vi "Data-DCSL__RecursionCtl.vi"(8 "TEMP DONT LINE":cluster{"LabelPath":string, "Ref":refnum<vi>}[](array[cluster]), 11 "Controls[] input":cluster{"LabelPath":string, "Ref":refnum<vi>}[](array[cluster])) -> (3 "Controls[] output":cluster{"LabelPath":string, "Ref":refnum<vi>}[](array[cluster]))   [LabVIEW 2017]
doc: "<B>#yyll</B>\nGetAllRefsByRecursion"
panel:
  # "递归了\nRadio Buttons（感觉没必要）\nCluster\nTab Control\n\n没递归\n数组"
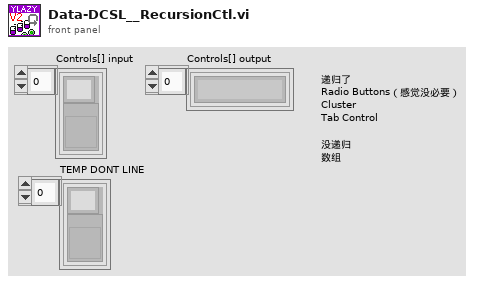
[diagram p1: front panel]
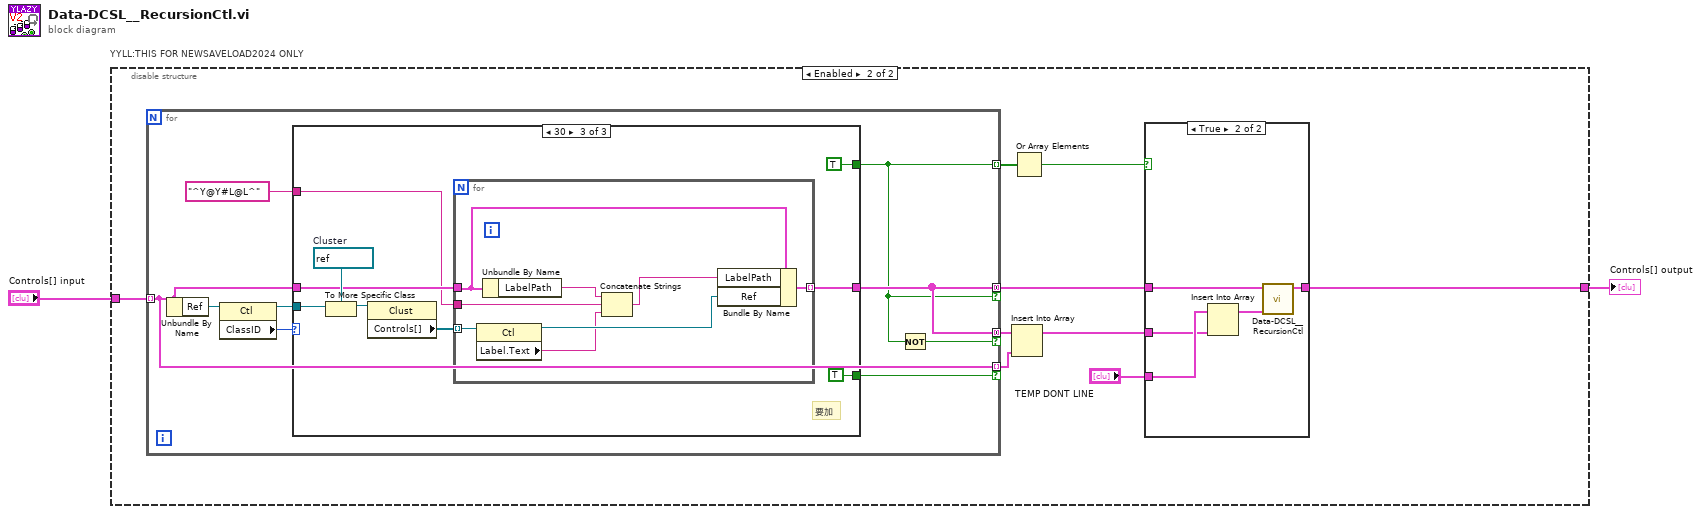
[diagram p0: block diagram]
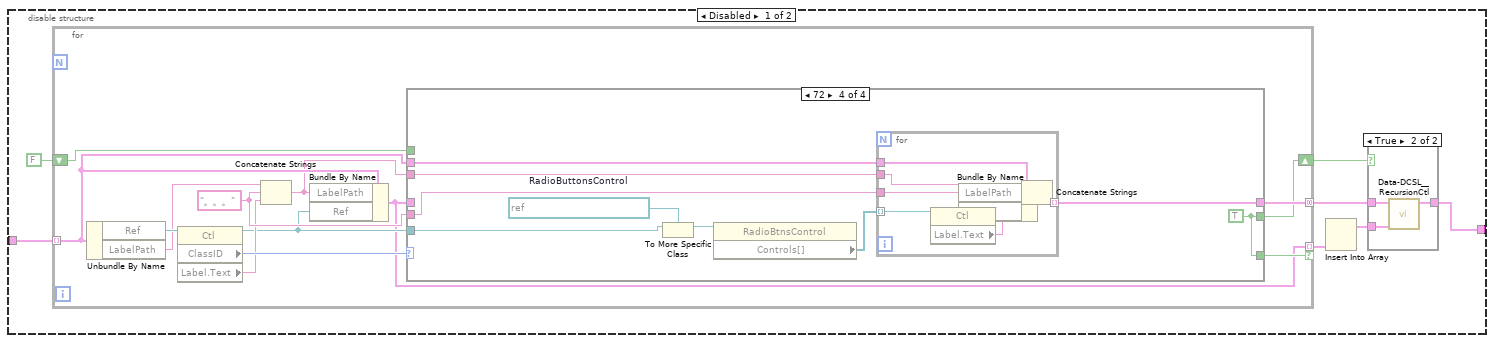
[diagram p2: hidden frame]
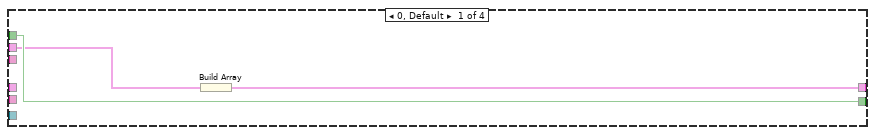
[diagram p3: hidden frame]
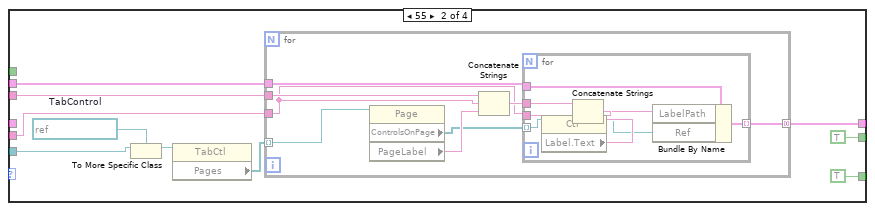
[diagram p4: hidden frame]
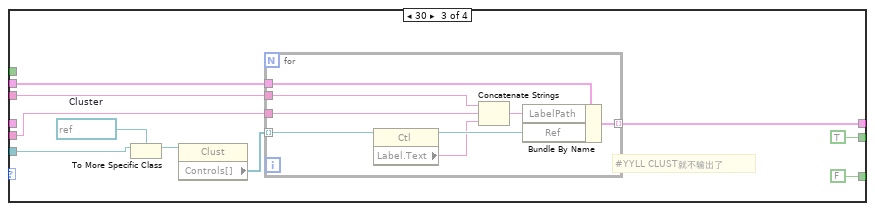
[diagram p5: hidden frame]
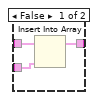
[diagram p6: hidden frame]
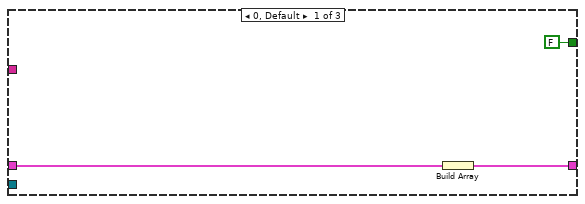
[diagram p7: hidden frame]
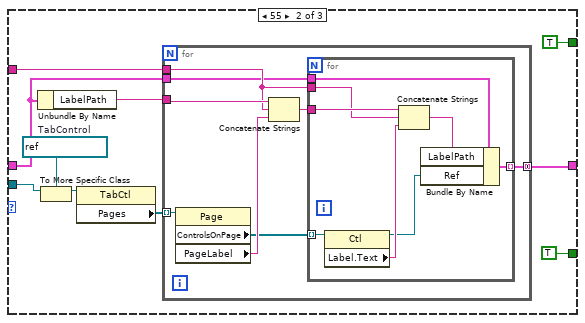
[diagram p8: hidden frame]
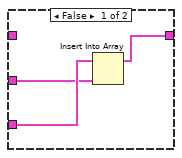
[diagram p9: hidden frame]
diagram:
  n1 = disable-structure "YYLL:THIS FOR NEWSAVELOAD2024 ONLY" shown="Enabled" {
    disable-tunnel: [w9 w97] -> w2
    disable-tunnel: "Controls[] input" -> [w8 w101]
    frame Disabled {
      n2 = for {
        tunnel: [w22] -> w7 mode=concatenating
        tunnel: w8 -> [w13] mode=indexing
        tunnel: [w11] -> w3 mode=indexing if=w18
        shift-right: [w21] -> w4
        shift-left: FALSE -> [w20]
        w15 = "。。。" ("string")
        n3 = Unbundle By Name(w13) -> ("Ref"=w17:refnum<vi>, "LabelPath"=w16:string)
        n4 = property class="Ctl"(reference=w17) -> (reference out=w12:refnum<vi>, "ClassID"=w19:u32, "Label.Text"=w14:string)  [unwired: 1 in, 1 out]
        n5 = Concatenate Strings(w16, w15, w14) -> (w10:string)
        n6 = Bundle By Name(cluster=w13, "LabelPath"=w10, "Ref"=w12) -> (w11:cluster{"LabelPath":string, "Ref":refnum<vi>})
        n7 = case shown="72" w19 {
          tunnel: w12 -> [_ w32 w60 w76]
          tunnel: [w25 w31 w54 w71] -> w22
          tunnel: [w24 TRUE TRUE w78] -> w21
          tunnel: w20 -> [w24 _ _ _]
          tunnel: [_ TRUE FALSE w78] -> w18
          tunnel: w13 -> [w23 w28 w56 w73]
          tunnel: w15 -> [_ w29 w55 w72]
          tunnel: w11 -> [_ _ _ _]
          tunnel: w10 -> [_ w26 w52 w70]
          frame 0, Default {
            n8 = Build Array(w23) -> (w25:cluster{"LabelPath":string, "Ref":refnum<vi>}[])
          }
          frame 55 {
            w35 = refnum<vi> refnum  # TabControl
            n9 = To More Specific Class(target class=w35, reference=w32) -> (specific class reference=w34:refnum<vi>)  [unwired: 1 in, 1 out]
            n10 = property class="TabCtl"(reference=w34) -> ("Pages"=w33:refnum<vi>[])  [unwired: 1 in, 2 out]
            n11 = for {
              tunnel: w33 -> [w43] mode=indexing
              tunnel: [w36] -> w31 mode=concatenating
              tunnel: w26 -> [w42]
              tunnel: w29 -> [w38]
              tunnel: w28 -> [w37]
              n12 = property class="Page"(reference=w43) -> ("ControlsOnPage"=w40:refnum<vi>[], "PageLabel"=w41:string)  [unwired: 1 in, 2 out]
              n13 = Concatenate Strings(w42, w38, w41) -> (w39:string)
              n14 = for {
                tunnel: w40 -> [w51] mode=indexing
                tunnel: w39 -> [w49]
                tunnel: w38 -> [w48]
                tunnel: w37 -> [w47]
                tunnel: [w44] -> w36 mode=indexing
                n15 = property class="Ctl"(reference=w51) -> (reference out=w45:refnum<vi>, "Label.Text"=w50:string)  [unwired: 1 in, 1 out]
                n16 = Concatenate Strings(w49, w48, w50) -> (w46:string)
                n17 = Bundle By Name(cluster=w47, "LabelPath"=w46, "Ref"=w45) -> (w44:cluster{"LabelPath":string, "Ref":refnum<vi>})
              }
            }
          }
          frame 30 {
            w61 = refnum<vi> refnum  # Cluster
            # "#YYLL CLUST就不输出了"
            n18 = To More Specific Class(target class=w61, reference=w60) -> (specific class reference=w59:refnum<vi>)  [unwired: 1 in, 1 out]
            n19 = property class="Clust"(reference=w59) -> ("Controls[]"=w57:refnum<vi>[])  [unwired: 1 in, 2 out]
            n20 = for {
              tunnel: w57 -> [w68] mode=indexing
              tunnel: w56 -> [w69]
              tunnel: w52 -> [w66]
              tunnel: w55 -> [w65]
              tunnel: [w62] -> w54 mode=indexing
              n21 = property class="Ctl"(reference=w68) -> (reference out=w64:refnum<vi>, "Label.Text"=w63:string)  [unwired: 1 in, 1 out]
              n22 = Concatenate Strings(w66, w65, w63) -> (w67:string)
              n23 = Bundle By Name(cluster=w69, "LabelPath"=w67, "Ref"=w64) -> (w62:cluster{"LabelPath":string, "Ref":refnum<vi>})
            }
          }
          frame 72 {
            w77 = refnum<vi> refnum  # RadioButtonsControl
            w78 = TRUE
            n24 = To More Specific Class(target class=w77, reference=w76) -> (specific class reference=w75:refnum<vi>)  [unwired: 1 in, 1 out]
            n25 = property class="RadioBtnsControl"(reference=w75) -> ("Controls[]"=w74:refnum<vi>[])  [unwired: 1 in, 2 out]
            n26 = for {
              tunnel: w74 -> [w85] mode=indexing
              tunnel: w73 -> [w86]
              tunnel: w70 -> [w83]
              tunnel: w72 -> [w82]
              tunnel: [w79] -> w71 mode=indexing
              n27 = property class="Ctl"(reference=w85) -> (reference out=w81:refnum<vi>, "Label.Text"=w80:string)  [unwired: 1 in, 1 out]
              n28 = Concatenate Strings(w83, w82, w80) -> (w84:string)
              n29 = Bundle By Name(cluster=w86, "LabelPath"=w84, "Ref"=w81) -> (w79:cluster{"LabelPath":string, "Ref":refnum<vi>})
            }
          }
        }
      }
      n30 = Insert Into Array(new element=w3) -> (w6:cluster{"LabelPath":string, "Ref":refnum<vi>}[])  [unwired: 2 in]
      n31 = case shown="True" w4 {
        tunnel: w7 -> [w89 w92]
        tunnel: [w88 w91] -> w9
        tunnel: w6 -> [w87 w90]
        frame False {
          n32 = Insert Into Array(array=w89, new element=w87) -> (w88:cluster{"LabelPath":string, "Ref":refnum<vi>}[])  [unwired: 1 in]
        }
        frame True {
          n33 = call "Data-DCSL__RecursionCtl.vi"("TEMP DONT LINE"=w90, "Controls[] input"=w92) -> ("Controls[] output"=w91:cluster{"LabelPath":string, "Ref":refnum<vi>}[])  [unwired: 9 in]
        }
      }
    }
    frame Enabled {
      n34 = for {
        tunnel: w101 -> [w103] mode=indexing
        tunnel: [w106] -> w100 mode=indexing
        tunnel: [w107] -> w98 mode=concatenating if=w106
        tunnel: [w107] -> w95 mode=concatenating if=w105
        tunnel: [w103] -> w93 mode=indexing if=w102
        n35 = Unbundle By Name(w103) -> ("Ref"=w110:refnum<vi>)
        n36 = property class="Ctl"(reference=w110) -> (reference out=w108:refnum<vi>, "ClassID"=w109:u32)  [unwired: 1 in, 1 out]
        n37 = case shown="30" w109 {
          tunnel: w108 -> [_ w120 w145]
          tunnel: [FALSE TRUE TRUE] -> w106
          tunnel: w103 -> [w112 w116 w143]
          tunnel: [w111 w115 w141] -> w107
          tunnel: "^Y@Y#L@L^" ("string") -> [_ w117 w142]
          tunnel: [_ TRUE TRUE] -> w102
          frame 0, Default {
            n38 = Build Array(w112) -> (w111:cluster{"LabelPath":string, "Ref":refnum<vi>}[])
          }
          frame 55 {
            w121 = refnum<vi> refnum  # TabControl
            n39 = Unbundle By Name(w116) -> ("LabelPath"=w118:string)
            n40 = To More Specific Class(target class=w121, reference=w120) -> (specific class reference=w122:refnum<vi>)  [unwired: 1 in, 1 out]
            n41 = property class="TabCtl"(reference=w122) -> ("Pages"=w119:refnum<vi>[])  [unwired: 1 in, 2 out]
            n42 = for {
              tunnel: w119 -> [w131] mode=indexing
              tunnel: w118 -> [w130]
              tunnel: w117 -> [w126]
              tunnel: w116 -> [w125]
              tunnel: [w124] -> w115 mode=concatenating
              n43 = property class="Page"(reference=w131) -> ("ControlsOnPage"=w128:refnum<vi>[], "PageLabel"=w129:string)  [unwired: 1 in, 2 out]
              n44 = Concatenate Strings(w130, w126, w129) -> (w127:string)
              n45 = for {
                tunnel: w128 -> [w139] mode=indexing
                tunnel: w127 -> [w138]
                tunnel: w126 -> [w137]
                tunnel: w125 -> [w135]
                tunnel: [w132] -> w124 mode=indexing
                n46 = property class="Ctl"(reference=w139) -> (reference out=w133:refnum<vi>, "Label.Text"=w136:string)  [unwired: 1 in, 1 out]
                n47 = Concatenate Strings(w138, w137, w136) -> (w134:string)
                n48 = Bundle By Name(cluster=w135, "LabelPath"=w134, "Ref"=w133) -> (w132:cluster{"LabelPath":string, "Ref":refnum<vi>})
              }
            }
          }
          frame 30 {
            w146 = refnum<vi> refnum  # Cluster
            # "要加"
            n49 = To More Specific Class(target class=w146, reference=w145) -> (specific class reference=w147:refnum<vi>)  [unwired: 1 in, 1 out]
            n50 = property class="Clust"(reference=w147) -> ("Controls[]"=w144:refnum<vi>[])  [unwired: 1 in, 2 out]
            n51 = for {
              tunnel: w144 -> [w156] mode=indexing
              tunnel: w143 -> [w155]
              tunnel: w142 -> [w151]
              tunnel: [w149] -> w141 mode=indexing
              n52 = property class="Ctl"(reference=w156) -> (reference out=w154:refnum<vi>, "Label.Text"=w152:string)  [unwired: 1 in, 1 out]
              n53 = Unbundle By Name(w155) -> ("LabelPath"=w153:string)
              n54 = Concatenate Strings(w153, w151, w152) -> (w150:string)
              n55 = Bundle By Name(cluster=w155, "LabelPath"=w150, "Ref"=w154) -> (w149:cluster{"LabelPath":string, "Ref":refnum<vi>})
            }
          }
        }
        n56 = Not(x=w106) -> (.not. x?=w105:bool)
      }
      n57 = Insert Into Array(array=w95, new element=w93) -> (w94:cluster{"LabelPath":string, "Ref":refnum<vi>}[])  [unwired: 1 in]
      n58 = Or Array Elements(Boolean array=w100) -> (logical OR=w99:bool)
      n59 = case shown="True" w99 {
        tunnel: w98 -> [_ w164]
        tunnel: [w157 w163] -> w97
        tunnel: "TEMP DONT LINE" -> [w159 w161]
        tunnel: w94 -> [w158 w160]
        frame False {
          n60 = Insert Into Array(array=w159, new element=w158) -> (w157:cluster{"LabelPath":string, "Ref":refnum<vi>}[])  [unwired: 1 in]
        }
        frame True {
          n61 = Insert Into Array(array=w161, new element=w160) -> (w162:cluster{"LabelPath":string, "Ref":refnum<vi>}[])  [unwired: 1 in]
          n62 = call "Data-DCSL__RecursionCtl.vi"("TEMP DONT LINE"=w162, "Controls[] input"=w164) -> ("Controls[] output"=w163:cluster{"LabelPath":string, "Ref":refnum<vi>}[])  [unwired: 9 in]
        }
      }
    }
  }
  "Controls[] output" <- w2
